vi "Find Re-entrant VIs in Folder.vi"(8 "error in (no error)":errorcluster, 10 "Pattern":string[](array[string])=["*.vi"], 11 "Directory Path":path) -> (0 "error out":errorcluster, 3 "VI List":path[](array[path]))   [LabVIEW 2016, in "SLL Scripting.lvlib"]
doc: "This VI can be used to find the list of re-entrant VIs in a folder."
uses:
  SLL Scripting.lvlib
panel:
  out "Progress":i32
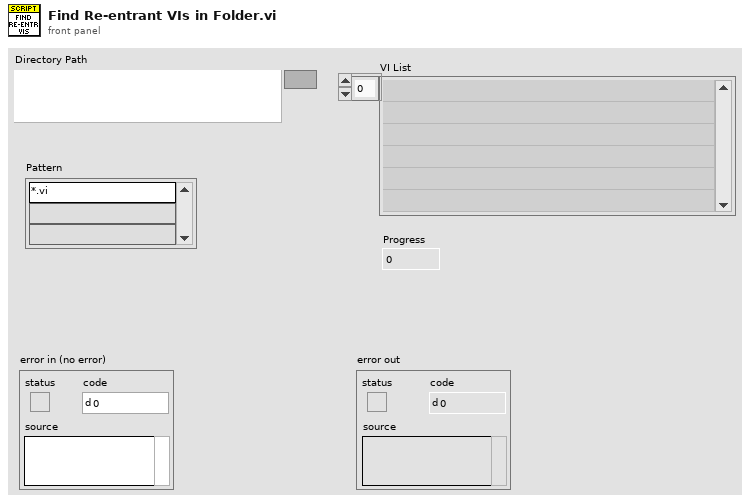
[diagram p1: front panel]
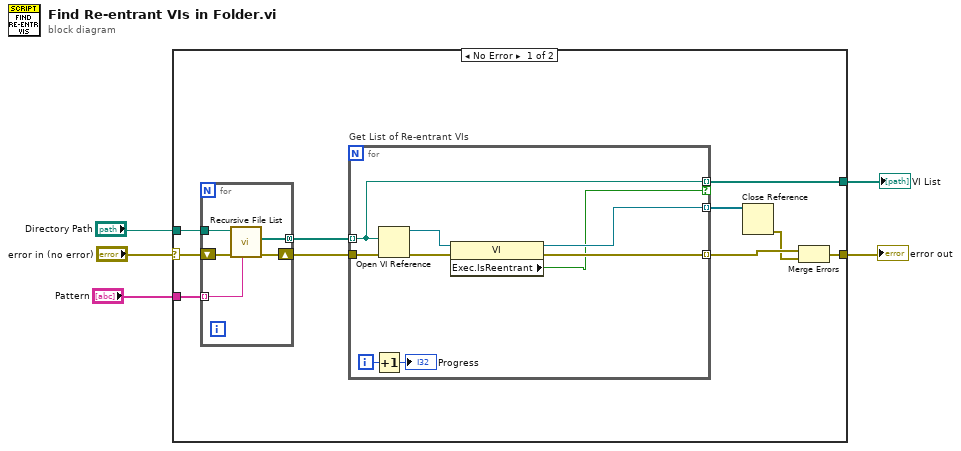
[diagram p0: block diagram]
diagram:
  n1 = case shown="No Error" "error in (no error)" {
    selector: "error in (no error)" -> [w11 w30]
    tunnel: "Directory Path" -> [w14 _]
    tunnel: [w12 _] -> w4
    tunnel: [w7 w30] -> w2
    tunnel: "Pattern" -> [w6 _]
    frame No Error {
      n2 = for {
        tunnel: w14 -> [w20]
        tunnel: [w19] -> w13 mode=concatenating
        shift-right: [w17] -> w10
        shift-left: w11 -> [w18]
        tunnel: w6 -> [w16] mode=indexing
        n3 = call <vilib>:"Recursive File List.vi"("pattern"=w16, "error in (no error)"=w18, "Folder Path"=w20) -> ("error out"=w17:errorcluster, "All Files in Dir"=w19:path[])  [unwired: 4 in, 3 out]
      }
      n4 = for "Get List of Re-entrant VIs" {
        tunnel: [w28] -> w15 mode=indexing
        tunnel: w13 -> [w27] mode=indexing
        tunnel: [w27] -> w12 mode=indexing if=w22
        tunnel: w10 -> [w26]
        tunnel: [w24] -> w9 mode=indexing
        i -> [w23]
        n5 = Increment(x=w23) -> (x+1=→"Progress":i32)
        n6 = Open VI Reference(vi path=w27, error in (no error)=w26) -> (vi reference=w29:refnum<vi>, error out=w25:errorcluster)  [unwired: 4 in]
        n7 = property class="VI"(reference=w29, error in=w25) -> (reference out=w28:refnum<vi>, error out=w24:errorcluster, "Exec.IsReentrant"=w22:bool)
      }
      n8 = Close Reference(reference=w15) -> (error out=w8:errorcluster)  [unwired: 1 in]
      n9 = Merge Errors(w9, w8) -> (w7:errorcluster)
    }
    frame Error {
    }
  }
  "error out" <- w2
  "VI List" <- w4
